vi "CompVisionUtil_EstimateFieldToCamera.vi"(9 "FieldToTarget":T1={"Translation3d"={"X"=0.0, "Y"=0.0, "Z"=0.0}, "Rotation3d"={"Q_quaternion"={"R"=1.0, "V"=[0.0, 0.0, 0.0]}}} {"Translation3d"."Z" format="%14.3f"; "Translation3d"."Y" format="%14.3f"; "Translation3d"."X" format="%14.3f"}, 11 "CameraToTarget":T5={"TRANSLATION3D"={"X"=0.0, "Y"=0.0, "Z"=0.0}, "ROTATION3D"={"Q_quaternion"={"R"=1.0, "V"=[0.0, 0.0, 0.0]}}, "XF"=FALSE} {"TRANSLATION3D"."Z" format="%14.3f"; "TRANSLATION3D"."Y" format="%14.3f"; "TRANSLATION3D"."X" format="%14.3f"}) -> (3 "EstimateFieldToCamera":T1={"Translation3d"={"X"=0.0, "Y"=0.0, "Z"=0.0}, "Rotation3d"={"Q_quaternion"={"R"=1.0, "V"=[0.0, 0.0, 0.0]}}} {"Translation3d"."Z" format="%14.3f"; "Translation3d"."Y" format="%14.3f"; "Translation3d"."X" format="%14.3f"})   [LabVIEW 2019, in "Trajectory_Library.lvlib"]
doc: "Estimates the pose of the camera in the field coordinate system, given the position of the target relative to the camera, and the target relative to the field. This *only* tracks the position of the camera, not the position of the robot itself.\n\nInputs:\n -- CameraToTarget -- Transform3d containing the position of the target relative to the camera.\n -- FieldToTarget -- Pose3d containing the position of the target in the field.\n\nOutput:\n -- EstimateFieldToCamera -- Pose3d containing position of the camera in the field."
uses:
  Trajectory_Library.lvlib
  TypeDef/TRANSLATION3D.ctl
  TypeDef/QUATERNION.ctl
  TypeDef/ROTATION3D.ctl
  TypeDef/TRANSFORM3D.ctl
  TypeDef/POSE3D.ctl
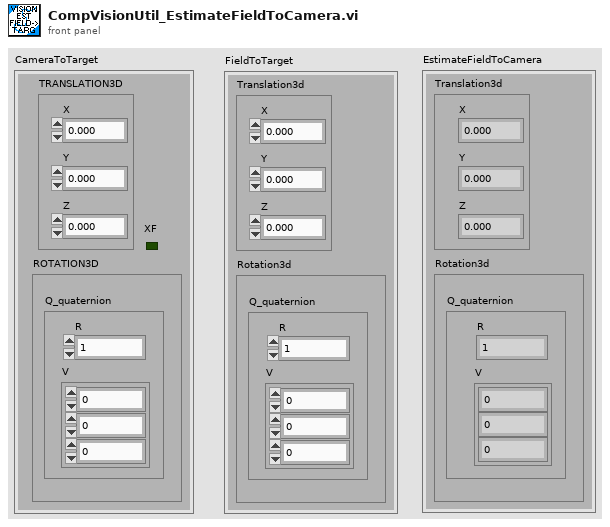
[diagram p1: front panel]
types:
  T1 = typedef "Trajectory_Library.lvlib/POSE3D.ctl" = cluster{"Translation3d":T2, "Rotation3d":T3}
  T2 = typedef "Trajectory_Library.lvlib/TRANSLATION3D.ctl" = cluster{"X":dbl, "Y":dbl, "Z":dbl}
  T3 = typedef "Trajectory_Library.lvlib/ROTATION3D.ctl" = cluster{"Q_quaternion":T4}
  T4 = typedef "Trajectory_Library.lvlib/QUATERNION.ctl" = cluster{"R":dbl, "V":dbl[]}
  T5 = typedef "Trajectory_Library.lvlib/TRANSFORM3D.ctl" = cluster{"TRANSLATION3D":T2, "ROTATION3D":T3, "XF":bool}
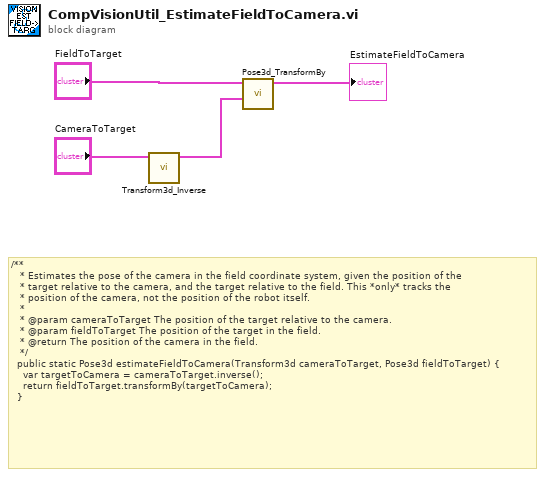
[diagram p0: block diagram]
diagram:
  # "/**\n   * Estimates the pose of the camera in the field coordinate system, given the position of the\n   * target relative to the camera, and the target relative to the field. This *only* tracks the\n   * position of the camera, not the position of the robot itself.\n   *\n   * @param cameraToTarget The position of the target relative to the camera.\n   * @param fieldToTarget The position of the target in the field.\n   * @return The position of the camera in the field.\n   */\n  public static Pose3d estimateFieldToCamera(Transform3d cameraToTarget, Pose3d fieldToTarget) {\n    var targetToCamera = cameraToTarget.inverse();\n    return fieldToTarget.transformBy(targetToCamera);\n  }"
  n1 = call "Transform3d_Inverse.vi"("inTransform3d"="CameraToTarget") -> ("outTransform3d"=w2:T5)  [unwired: 10 in]
  n2 = call "Pose3d_TransformBy.vi"("other Transform3d"=w2, "in Pose3d"="FieldToTarget") -> ("out POSE3d"=→"EstimateFieldToCamera":T1)  [unwired: 9 in]
